vi "test prompt without arguments.vi"(8 "error in (no error)":errorcluster) -> (0 "error out":errorcluster, 3 "body":string)   [LabVIEW 2020, in "MCP Server tests.lvlib"]
doc: "arguments is optional in prompts/get. A prompt that has no required arguments must be returned when the request has no arguments member."
uses:
  MCP Server tests.lvlib
  <vilib>/JDP Science/JSONtext/Next JSON Value.vi
  <vilib>/JDP Science/JSONtext/String Subset.vi
  <vilib>/JDP Science/JSONtext/Parsing/Advance past next JSON Value (inlined COPY).vi
  <vilib>/JDP Science/JSONtext/Parsing/Advance past whitespace.vi
  <vilib>/JDP Science/JSONtext/Parsing/Advance past String.vi
  <vilib>/JDP Science/JSONtext/Parsing/Advance past Number.vi
  <vilib>/JDP Science/JSONtext/Parsing/Advance past Line Ending.vi
  <vilib>/JDP Science/JSONtext/Parsing/Parse Full Path or Item Name.vi
  <vilib>/JDP Science/JSONtext/Parsing/Advance past Array.vi
  <vilib>/JDP Science/JSONtext/Parsing/Advance past Object.vi
  <vilib>/JDP Science/JSONtext/support/Error Cluster From Code.vi
  <vilib>/JDP Science/JSONtext/Offset/Find Item Locations by Path.vi
  <vilib>/addons/_JKI Toolkits/Caraya/classes/Test/Test.lvclass
  <vilib>/JDP Science/JSONtext/JSONtext.lvlib
  <vilib>/addons/_JKI Toolkits/Caraya/classes/Assert/Assert.lvclass
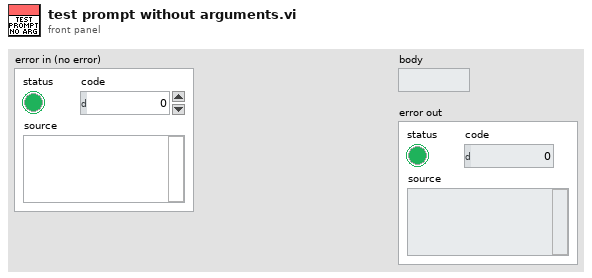
[diagram p1: front panel]
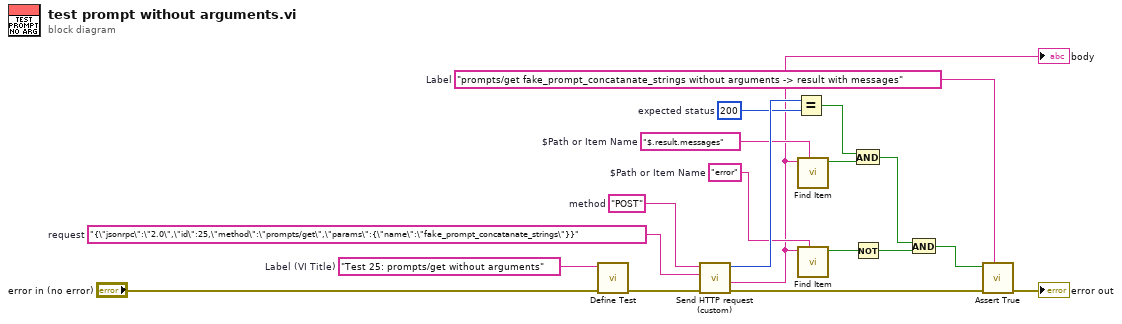
[diagram p0: block diagram]
diagram:
  w3 = "prompts/get fake_prompt_concatanate_strings without arguments -> result with messages"  # Label
  w11 = "error"  # $Path or Item Name
  w12 = "$.result.messages"  # $Path or Item Name
  w13 = 200  # expected status
  w16 = "{\"jsonrpc\":\"2.0\",\"id\":25,\"method\":\"prompts/get\",\"params\":{\"name\":\"fake_prompt_concatanate_strings\"}}"  # request
  w17 = "POST"  # method
  w19 = "Test 25: prompts/get without arguments"  # Label (VI Title)
  n1 = call <vilib>:"Define Test.vi"("error in (no error)"="error in (no error)", "Label (VI Title)"=w19) -> ("error out"=w15:errorcluster)  [unwired: 8 in, 1 out]
  n2 = call "Send HTTP request (custom).vi"("error in (no error)"=w15, "request"=w16, "method"=w17) -> ("error out"=w4:errorcluster, "response"=w2:string, "status code"=w14:i32)  [unwired: 5 in, 1 out]
  "body" <- w2
  n3 = Equal?(x=w14, y=w13) -> (x = y?=w9:bool)
  n4 = call <vilib>:"Find Item.vi"("$Path or Item Name"=w12, "JSON"=w2) -> ("Found"=w8:bool)  [unwired: 6 in, 3 out]
  n5 = call <vilib>:"Find Item.vi"("$Path or Item Name"=w11, "JSON"=w2) -> ("Found"=w10:bool)  [unwired: 6 in, 3 out]
  n6 = And(x=w9, y=w8) -> (x .and. y?=w7:bool)
  n7 = Not(x=w10) -> (.not. x?=w6:bool)
  n8 = And(x=w7, y=w6) -> (x .and. y?=w5:bool)
  n9 = call <vilib>:"Assert True.vi"("Label"=w3, "error in (no error)"=w4, "True?"=w5) -> ("error out"=→"error out":errorcluster)  [unwired: 7 in, 1 out]
